vi "DAC Save Results.vi"(8 "error in":errorcluster, 9 "Log Details?":bool, 10 "tdms file":refnum<k34>, 11 "DAC Jumo DP in":refnum<class "DAC Jumo DP.lvclass">) -> (0 "error out":errorcluster)   [LabVIEW 2019, in "DAC.lvlib" / "DAC Jumo DP.lvclass"]
uses:
  DAC Jumo DP.lvclass
  C:/Users/wg/Documents/LV_Projects/test-stand/App/DAC/DAC.lvclass
  DAC.lvclass/DAC.ctl
  DAC Jumo DP.lvclass/DAC Jumo DP.ctl
  DAC.lvclass
  <vilib>/Analysis/NI_AALBase.lvlib
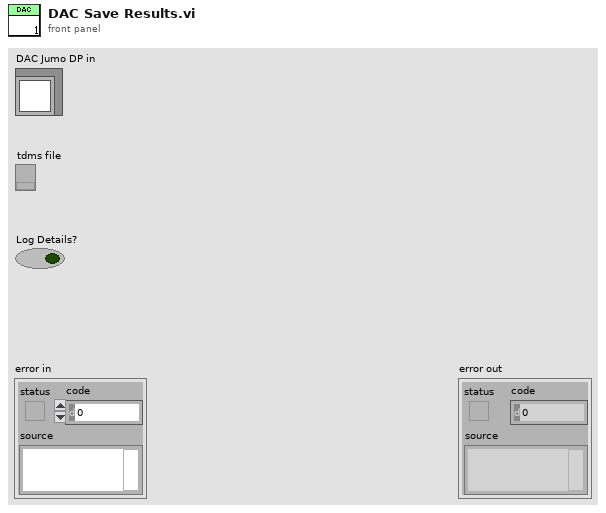
[diagram p1: front panel]
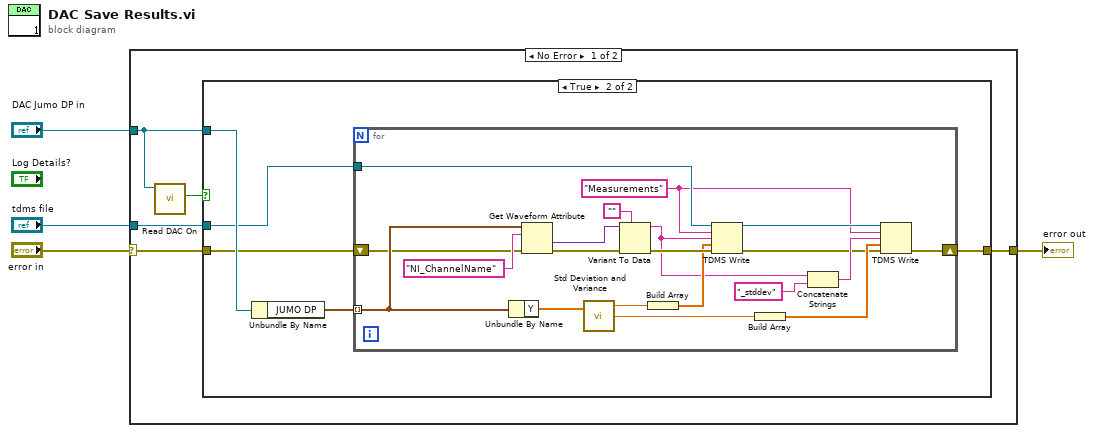
[diagram p0: block diagram]
diagram:
  n1 = case shown="No Error" "error in" {
    selector: "error in" -> [w6 w36]
    tunnel: "DAC Jumo DP in" -> [w9 _]
    tunnel: "tdms file" -> [w7 _]
    tunnel: [w5 w36] -> w1
    frame No Error {
      n2 = call "Read DAC On.vi"("DAC in"=w9) -> ("DAC On"=w8:bool)  [unwired: 8 in, 2 out]
      n3 = case shown="True" w8 {
        tunnel: w9 -> [_ w15]
        tunnel: w7 -> [_ w14]
        tunnel: w6 -> [w10 w12]
        tunnel: [w10 w11] -> w5
        frame False {
        }
        frame True {
          n4 = Unbundle By Name(w15) -> ("JUMO DP"=w13:waveform(dbl)[])
          n5 = for {
            tunnel: w14 -> [w35]
            tunnel: w13 -> [w31] mode=indexing
            shift-right: [w27] -> w11
            shift-left: w12 -> [w30]
            w19 = "Measurements" ("group name in (Untitled)")
            n6 = Unbundle By Name(w31) -> ("Y"=w23:dbl[])
            n7 = Get Waveform Attribute(4:w30, 6:"NI_ChannelName" ("name"), 7:w31) -> (0:w29:errorcluster, 1:w33:variant)  [unwired: 1 in, 2 out]
            n8 = call <vilib>:"Std Deviation and Variance.vi"("X"=w23) -> ("mean"=w26:dbl, "standard deviation"=w25:dbl)  [unwired: 1 in, 1 out]
            n9 = Variant To Data(error in=w29, type="", Variant=w33) -> (data=w21:string, error out=w28:errorcluster)
            n10 = Build Array(w26) -> (w22:dbl[])
            n11 = TDMS Write(0:w35, 5:w19, 7:w21, 9:w22, 11:w28) -> (4:w20:refnum<k34>, 15:w16:errorcluster)  [unwired: 1 in, 2 out]
            n12 = Build Array(w25) -> (w18:dbl[])
            n13 = Concatenate Strings(w21, "_stddev" ("string")) -> (w17:string)
            n14 = TDMS Write(0:w20, 5:w19, 7:w17, 9:w18, 11:w16) -> (15:w27:errorcluster)  [unwired: 1 in, 3 out]
          }
        }
      }
    }
    frame Error {
    }
  }
  "error out" <- w1
